vi "cycle_read.vi"() -> ()   [LabVIEW 2014]
uses:
  Map_lib/MapBuilder/Robot_Position.ctl
  <vilib>/Tufts CEEO ROS for LabVIEW Software/ROS/Code/Console/Servers/ServerSubs/TopicDef.ctl
  <vilib>/Tufts CEEO ROS for LabVIEW Software/ROS/Code/SubVIs/_ROSDirection.ctl
panel:
  out "Pose 2D":cluster{"x":dbl, "y":dbl, "theta":dbl}
  out "错误输出":errorcluster
  out "sensor_msg_cluster":cluster{"voltage":dbl, "motor":i8}
  out "robot_position_cluster":T1
  in  "stop2":bool
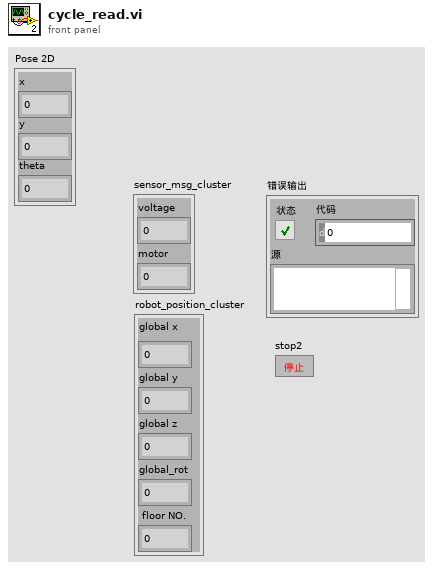
[diagram p1: front panel]
types:
  T1 = typedef "Robot_Position.ctl" = cluster{"global x":dbl, "global y":dbl, "global z":dbl, "global_rot":dbl, " floor NO.":dbl}
  T2 = typedef "TopicDef.ctl" = cluster{"Topic":string, "Type":string, "Action":T3, "Update (ms)":u16, "queue size":u16}
  T3 = typedef "_ROSDirection.ctl" = enum16{"Node", "Publisher", "Subscriber", "ServiceClient", "ServiceProvider"}
  T4 = typedef "_ROSControl.ctl" = cluster{"topic port":u16, "Node":string, "topic":string, "type":string, "node port":u16, "error ":errorcluster, "Direction":T3, "Update (ms)":u16, "FIFO size":u16}
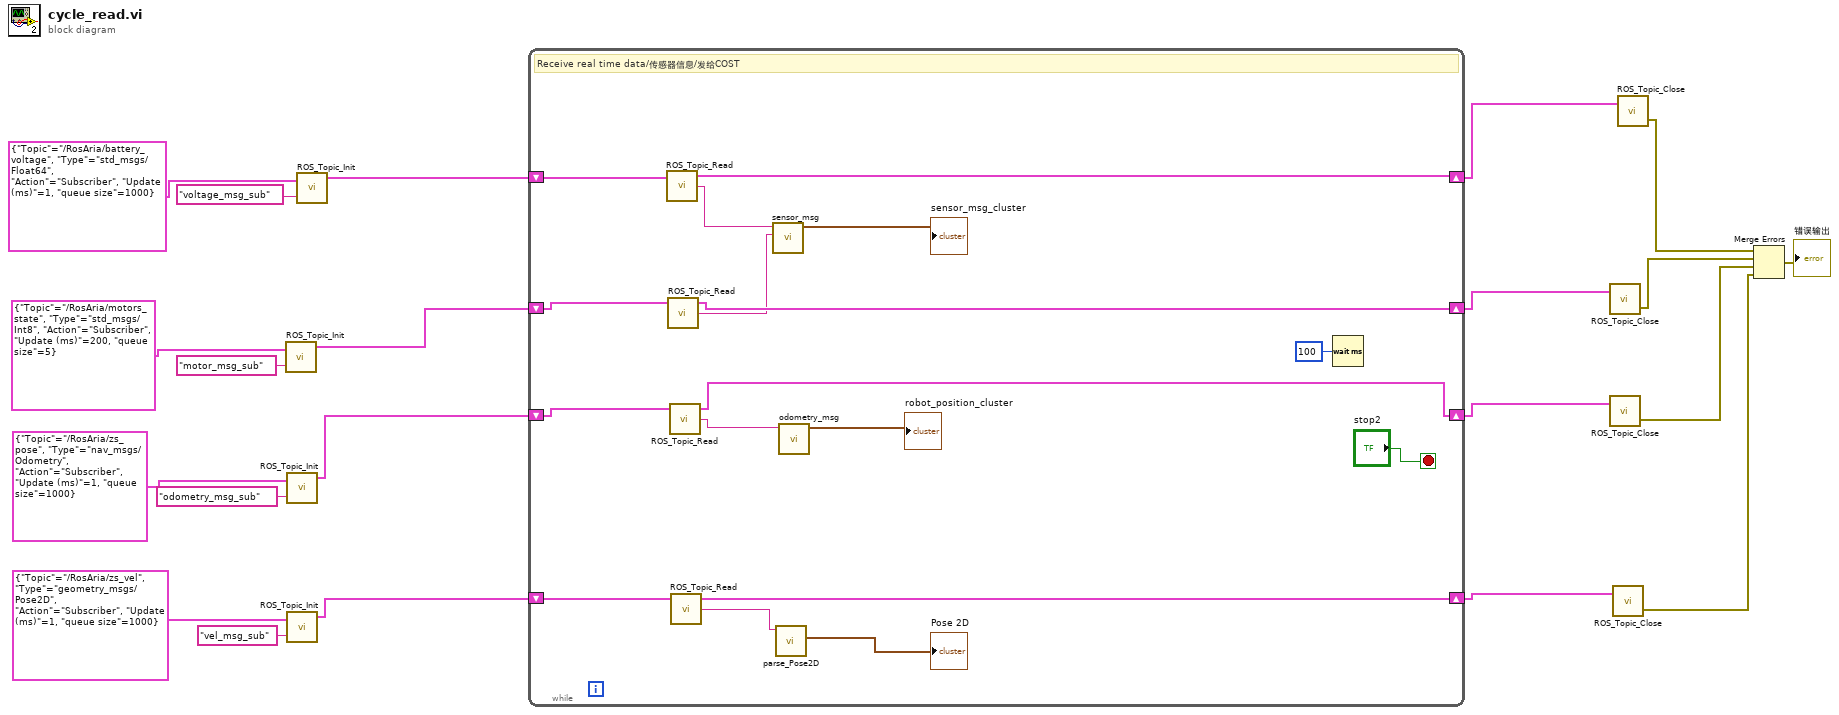
[diagram p0: block diagram]
diagram:
  n1 = call <vilib>:"ROS_Topic_Init.vi"("Definitions"=T2 {"Topic"="/RosAria/motors_state", "Type"="std_msgs/Int8", "Action"=enum."Subscriber", "Update (ms)"=200, "queue size"=5}, "node"="motor_msg_sub") -> ("ROS out"=w15:T4)  [unwired: 1 in, 1 out]
  n2 = call <vilib>:"ROS_Topic_Init.vi"("Definitions"=T2 {"Topic"="/RosAria/zs_pose", "Type"="nav_msgs/Odometry", "Action"=enum."Subscriber", "Update (ms)"=1, "queue size"=1000}, "node"="odometry_msg_sub") -> ("ROS out"=w11:T4)  [unwired: 1 in, 1 out]
  n3 = call <vilib>:"ROS_Topic_Init.vi"("Definitions"=T2 {"Topic"="/RosAria/zs_vel", "Type"="geometry_msgs/Pose2D", "Action"=enum."Subscriber", "Update (ms)"=1, "queue size"=1000}, "node"="vel_msg_sub") -> ("ROS out"=w3:T4)  [unwired: 1 in, 1 out]
  n4 = call <vilib>:"ROS_Topic_Init.vi"("Definitions"=T2 {"Topic"="/RosAria/battery_voltage", "Type"="std_msgs/Float64", "Action"=enum."Subscriber", "Update (ms)"=1, "queue size"=1000}, "node"="voltage_msg_sub") -> ("ROS out"=w17:T4)  [unwired: 1 in, 1 out]
  n5 = while {
    shift-right: [w36] -> w16
    shift-left: w17 -> [w37]
    shift-right: [w34] -> w14
    shift-left: w15 -> [w35]
    shift-right: [w32] -> w10
    shift-left: w11 -> [w33]
    shift-right: [w24] -> w2
    shift-left: w3 -> [w25]
    stop <- "stop2" stop-if-true
    # "Receive real time data/传感器信息/发给COST"
    n6 = call <vilib>:"ROS_Topic_Read.vi"("ROS in"=w37) -> ("Reply"=w31:string, "ROS out"=w36:T4)  [unwired: 2 in, 1 out]
    n7 = call <vilib>:"ROS_Topic_Read.vi"("ROS in"=w35) -> ("Reply"=w30:string, "ROS out"=w34:T4)  [unwired: 2 in, 1 out]
    n8 = call <vilib>:"ROS_Topic_Read.vi"("ROS in"=w33) -> ("Reply"=w29:string, "ROS out"=w32:T4)  [unwired: 2 in, 1 out]
    n9 = call <vilib>:"ROS_Topic_Read.vi"("ROS in"=w25) -> ("Reply"=w23:string, "ROS out"=w24:T4)  [unwired: 2 in, 1 out]
    n10 = call "sensor_msg.vi"("motor_msg in"=w30, "voltage_msg in"=w31) -> ("sensor_msg_cluster"=→"sensor_msg_cluster":cluster{"voltage":dbl, "motor":i8})  [unwired: 9 in]
    n11 = call <vilib>:"parse_Pose2D.vi"("msg in"=w23) -> ("Pose 2D"=→"Pose 2D":cluster{"x":dbl, "y":dbl, "theta":dbl})  [unwired: 4 in, 2 out]
    n12 = call "odometry_msg.vi"("odometry_msg in"=w29) -> ("robot_position_cluster"=→"robot_position_cluster":T1)  [unwired: 8 in, 2 out]
    n13 = Wait (ms)(milliseconds to wait=u32 100 ("等待时间（毫秒）")) -> ()  [unwired: 1 out]
  }
  n14 = call <vilib>:"ROS_Topic_Close.vi"("ROS in"=w14) -> ("error out"=w8:errorcluster)  [unwired: 3 in]
  n15 = call <vilib>:"ROS_Topic_Close.vi"("ROS in"=w10) -> ("error out"=w7:errorcluster)  [unwired: 3 in]
  n16 = call <vilib>:"ROS_Topic_Close.vi"("ROS in"=w2) -> ("error out"=w1:errorcluster)  [unwired: 3 in]
  n17 = call <vilib>:"ROS_Topic_Close.vi"("ROS in"=w16) -> ("error out"=w9:errorcluster)  [unwired: 3 in]
  n18 = Merge Errors(w9, w8, w7, w1) -> (→"错误输出":errorcluster)
